vi "SC Show Result.vi"(4 "error in (no error)":errorcluster, 8 "OK message":string="Done.", 9 "output":string, 10 "result":string, 11 "title":string) -> (0 "error out":errorcluster)   [LabVIEW 2023]
doc: "Shows the outcome of a systemcore-deploy command in a dialog: the title, a sentence for the RESULT word (OK message for OK and CHECKED_OUT), and the command's output."
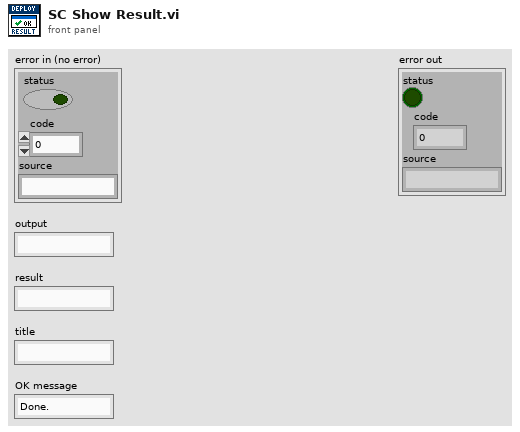
[diagram p1: front panel]
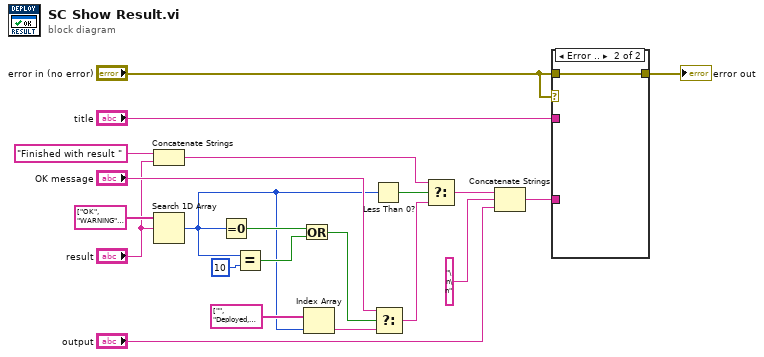
[diagram p0: block diagram]
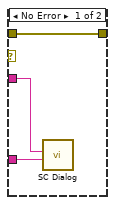
[diagram p2: hidden frame]
diagram:
  n1 = Concatenate Strings("Finished with result ", "result") -> (w9:string)
  n2 = Search 1D Array(1D array=string[] ["OK", "WARNING", "BROKEN", "UP_TO_DATE", "ERROR", "DIVERGED", "REPLACED", "MERGED", "UPDATED", "CURRENT", "CHECKED_OUT"], element="result") -> (index of element=w13:i32)  [unwired: 1 in]
  n3 = Equal To 0?(x=w13) -> (x = 0?=w18:bool)
  n4 = Equal?(x=w13, y=10) -> (x = y?=w17:bool)
  n5 = Or(x=w18, y=w17) -> (x .or. y?=w16:bool)
  n6 = Index Array(array=string[] ["", "Deployed, but with a warning (see below).", "The robot rejected the deploy because the entry VI is broken. The program that ran before keeps running.", "The robot already runs this; there was nothing to deploy.", "It didn't work (see below).", "Cancelled.", "The project now matches what the robot runs. The previous version is kept in git (see below).", "The robot's changes are merged into the project.", "The project now has the robot's changes (see below).", "The project already has everything the robot runs.", ""], index=w13) -> (element=w14:string)
  n7 = Less Than 0?(x=w13) -> (x < 0?=w10:bool)
  n8 = Select(t="OK message", s=w16, f=w14) -> (s? t:f=w8:string)
  n9 = Select(t=w9, s=w10, f=w8) -> (s? t:f=w7:string)
  n10 = Concatenate Strings(w7, "\n\n", "output") -> (w4:string)
  n11 = case shown="Error .." "error in (no error)" {
    tunnel: w4 -> [w24 _]
    tunnel: "error in (no error)" -> [w22 w25]
    tunnel: "title" -> [w23 _]
    tunnel: [w22 w25] -> w2
    frame No Error {
      n12 = call "SC Dialog.vi"("message"=w24, "window title"=w23) -> ()  [unwired: 9 in, 1 out]
    }
    frame Error {
    }
  }
  "error out" <- w2
